vi "AlliGator with Tabs Register Control Events.vi"(8 "Error In":errorcluster) -> (0 "Error Out":errorcluster, 3 "AlliGator Events Registration":T1)   [LabVIEW 2021, in "AlliGator GUI.lvlib"]
doc: "Registers user events for controls on the main AlliGator window."
uses:
  AlliGator GUI.lvlib
  Settings/AlliGator Settings+.lvlib
  Phasor Plot Color Map/AlliGator Phasor Plot Color Map.lvlib
  Graphs/XY Graph/XY Graph Add-Ons.lvlib
  Decay Graph/AlliGator Decay Graph.lvlib
  Intensity Time Trace/AlliGator Intensity Time Trace.lvlib
  Decay Statistics/AlliGator Decay Statistics.lvlib
  Phasor Graph/AlliGator Phasor Graph.lvlib
  Phasor Ratio/AlliGator Phasor Ratio.lvlib
  Lifetime & Other Parameters/AlliGator Lifetime & Other Parameters.lvlib
  Settings/AlliGator Settings Window Messages.ctl
  Settings/AlliGator Settings Event.ctl
  Phasor Plot Color Map/AlliGator Phasor Color Map User Event List.ctl
  AlliGator Subpanel Event Data.ctl
  Graphs/XY Graph/XY Graph Refnum.ctl
  AlliGator with Tabs Events Registration.ctl
  Phasor Plot/AlliGator Phasor Plot.lvlib
  Decay Fit Parameter Map/AlliGator Decay Fit Parameter Map.lvlib
  Parameter Map/AlliGator Parameter Map.lvlib
panel:
  # "see the AlliGator License on the block diagram (Ctrl+E or Window:Show Block Diagram)"
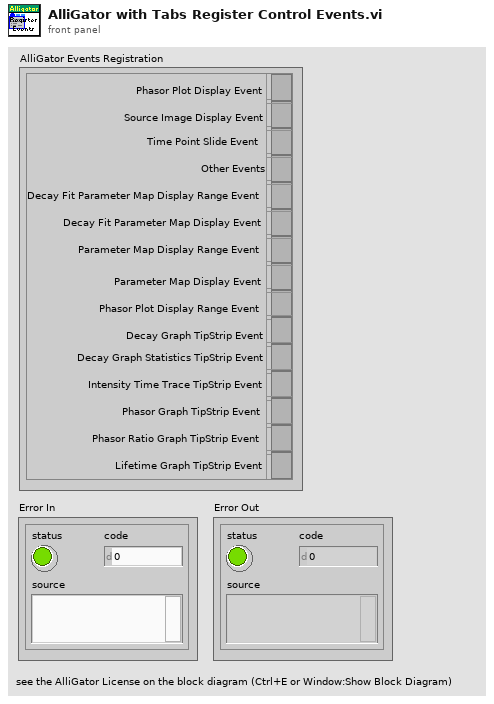
[diagram p1: front panel]
types:
  T1 = typedef "AlliGator GUI.lvlib/AlliGator with Tabs Events Registration.ctl" = cluster{"Phasor Plot Display Event":refnum<event-registration>, "Source Image Display Event":refnum<event-registration>, "Time Point Slide Event":refnum<event-registration>, "Other Events":refnum<event-registration>, "Decay Fit Parameter Map Display Range Event":refnum<event-registration>, "Decay Fit Parameter Map Display Event":refnum<event-registration>, "Parameter Map Display Range Event":refnum<event-registration>, "Parameter Map Display Event":refnum<event-registration>, "Phasor Plot Display Range Event":refnum<event-registration>, "Decay Graph TipStrip Event":refnum<event-registration>, "Decay Graph Statistics TipStrip Event":refnum<event-registration>, "Intensity Time Trace TipStrip Event":refnum<event-registration>, "Phasor Graph TipStrip Event":refnum<event-registration>, "Phasor Ratio Graph TipStrip Event":refnum<event-registration>, "Lifetime Graph TipStrip Event":refnum<event-registration>}
  T2 = typedef "AlliGator Decay Graph.lvlib/AlliGator Decay Graph Ctrl Refnums.ctl" = cluster{"Decay Graph":refnum<vi>, "Decay Graph Active":refnum<vi>, "Decay Background":refnum<vi>, "Decay Integrated Intensity":refnum<vi>, "Decay Lifetime":refnum<vi>}
  T3 = typedef "AlliGator Decay Statistics.lvlib/AlliGator Decay Statistics Graph Ctrl Refnums.ctl" = cluster{"Decay Statistics Graph":refnum<vi>, "Decay Statistics Bin":refnum<vi>}
  T4 = typedef "AlliGator Intensity Time Trace.lvlib/AlliGator Intensity Time Trace Ctrl Refnums.ctl" = cluster{"Intensity Time Trace":refnum<vi>, "Time Step":refnum<vi>, "Use File Timestamp":refnum<vi>}
  T5 = typedef "AlliGator Phasor Graph.lvlib/AlliGator Phasor Graph Ctrl Refnums.ctl" = cluster{"Phasor Ratio":refnum<vi>, "Modulus Lifetime":refnum<vi>, "Phasor at cursor (m, phi)":refnum<vi>, "Phase Lifetime":refnum<vi>, "Phasor at cursor (g, s)":refnum<vi>, "Phasor Graph Average Lifetime":refnum<vi>, "Phasor Graph Active":refnum<vi>, "Save Phasor Graph":refnum<vi>, "Phasor Frame Slide":refnum<vi>, "Single Step Phasor":refnum<vi>, "Calibration Type":refnum<vi>, "Show Line":refnum<vi>, "Phase Lifetime 1":refnum<vi>, "Phase Lifetime 2":refnum<vi>, "Phasor Graph Frequency":refnum<vi>, "Phasor Reference 1 Control":refnum<vi>, "Phasor Reference 2 Control":refnum<vi>, "Calibration Lifetime":refnum<vi>, "Phase Lifetime SDV":refnum<vi>, "Average Lifetime SDV":refnum<vi>, "Phasor Ratio SDV":refnum<vi>, "Modulus Lifetime SDV":refnum<vi>, "Phasor Graph":refnum<vi>}
  T6 = typedef "AlliGator Phasor Ratio.lvlib/AlliGator Phasor Ratio Graph Ctrl Refnums.ctl" = cluster{"Phasor Ratio Graph":refnum<vi>}
  T7 = typedef "AlliGator Lifetime & Other Parameters.lvlib/AlliGator Lifetime & Other Parameters Ctrl Refnums.ctl" = cluster{"Lifetime Graph":refnum<vi>}
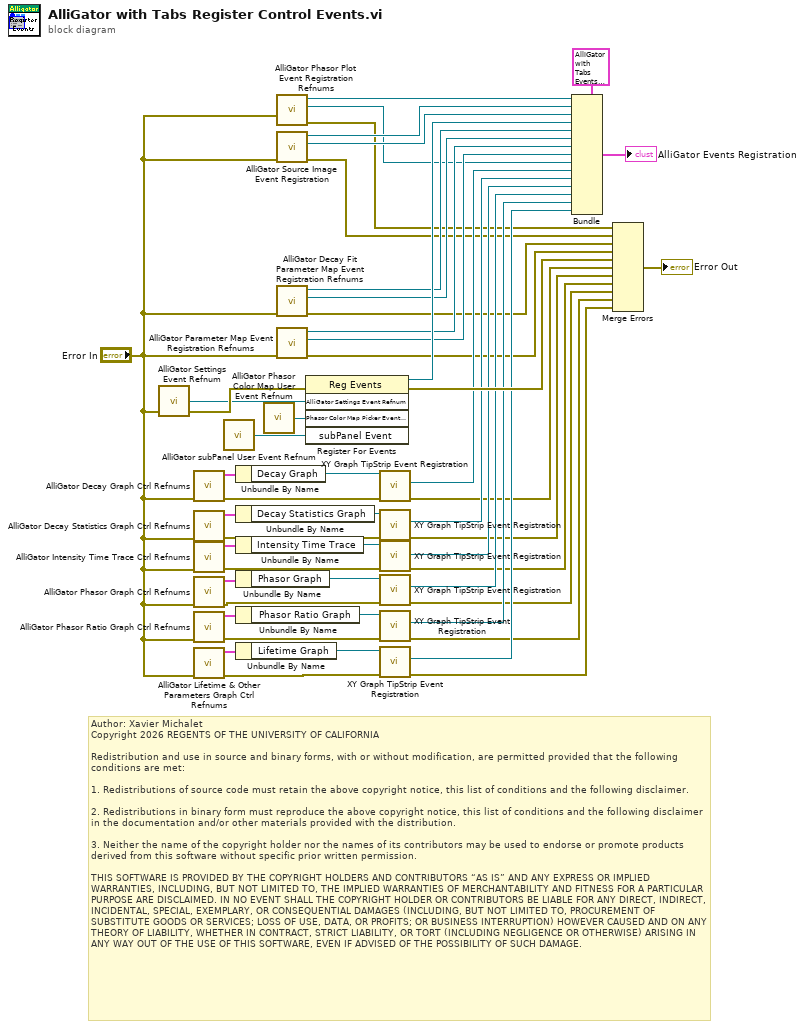
[diagram p0: block diagram]
diagram:
  # "Author: Xavier Michalet\nCopyright 2026 REGENTS OF THE UNIVERSITY OF CALIFORNIA\n\nRedistribution and use in source and binary forms, with or without modification, are permitted provided that the following conditions are met:\n\n1. Redistributions of source code must retain the above copyright notice, this list of conditions and the following disclaimer.\n\n2. Redistributions in binary form must reproduce the above copyright notice, this list of conditions and the following disclaimer in the documentation and/or other materials provided with the distribution.\n\n3. Neither the name of the copyright holder nor the names of its contributors may be used to endorse or promote products derived from this software without specific prior written permission.\n\nTHIS SOFTWARE IS PROVIDED BY THE COPYRIGHT HOLDERS AND CONTRIBUTORS “AS IS” AND ANY EXPRESS OR IMPLIED WARRANTIES, INCLUDING, BUT NOT LIMITED TO, THE IMPLIED WARRANTIES OF MERCHANTABILITY AND FITNESS FOR A PARTICULAR PURPOSE ARE DISCLAIMED. IN NO EVENT SHALL THE COPYRIGHT HOLDER OR CONTRIBUTORS BE LIABLE FOR ANY DIRECT, INDIRECT, INCIDENTAL, SPECIAL, EXEMPLARY, OR CONSEQUENTIAL DAMAGES (INCLUDING, BUT NOT LIMITED TO, PROCUREMENT OF SUBSTITUTE GOODS OR SERVICES; LOSS OF USE, DATA, OR PROFITS; OR BUSINESS INTERRUPTION) HOWEVER CAUSED AND ON ANY THEORY OF LIABILITY, WHETHER IN CONTRACT, STRICT LIABILITY, OR TORT (INCLUDING NEGLIGENCE OR OTHERWISE) ARISING IN ANY WAY OUT OF THE USE OF THIS SOFTWARE, EVEN IF ADVISED OF THE POSSIBILITY OF SUCH DAMAGE."
  n1 = call "AlliGator Settings Event Refnum.vi"("Error In"="Error In") -> ("AlliGator Settings Event Refnum"=w11:refnum<user-event>, "Error Out"=w45:errorcluster)  [unwired: 7 in]
  n2 = call "AlliGator Decay Graph Ctrl Refnums.vi"("error in (no error)"="Error In") -> ("error out"=w23:errorcluster, "Decay Graph Ctrl Refnums"=w35:T2)  [unwired: 9 in]
  n3 = call "AlliGator Decay Statistics Graph Ctrl Refnums.vi"("error in (no error)"="Error In") -> ("error out"=w22:errorcluster, "Decay Statistics Graph Ctrl Refnums"=w31:T3)  [unwired: 9 in]
  n4 = call "AlliGator Intensity Time Trace Ctrl Refnums.vi"("error in (no error)"="Error In") -> ("error out"=w21:errorcluster, "Intensity Time Trace Ctrl Refnums"=w33:T4)  [unwired: 9 in]
  n5 = call "AlliGator Phasor Graph Ctrl Refnums.vi"("error in (no error)"="Error In") -> ("error out"=w20:errorcluster, "Phasor Graph Ctrl Refnums"=w29:T5)  [unwired: 9 in]
  n6 = call "AlliGator Phasor Ratio Graph Ctrl Refnums.vi"("error in (no error)"="Error In") -> ("error out"=w19:errorcluster, "Phasor Ratio Graph Ctrl Refnums"=w27:T6)  [unwired: 9 in]
  n7 = call "AlliGator Lifetime & Other Parameters Graph Ctrl Refnums.vi"("error in (no error)"="Error In") -> ("error out"=w18:errorcluster, "Lifetime & Other Parameters Graph Ctrl Refnums"=w25:T7)  [unwired: 9 in]
  n8 = call "AlliGator subPanel User Event Refnum.vi"() -> ("subPanel Event"=w49:refnum<user-event>)  [unwired: 9 in]
  n9 = Unbundle By Name(w35) -> ("Decay Graph"=w34:refnum<vi>)
  n10 = Unbundle By Name(w31) -> ("Decay Statistics Graph"=w30:refnum<vi>)
  n11 = Unbundle By Name(w33) -> ("Intensity Time Trace"=w32:refnum<vi>)
  n12 = Unbundle By Name(w29) -> ("Phasor Graph"=w28:refnum<vi>)
  n13 = Unbundle By Name(w27) -> ("Phasor Ratio Graph"=w26:refnum<vi>)
  n14 = Unbundle By Name(w25) -> ("Lifetime Graph"=w24:refnum<vi>)
  n15 = call "AlliGator Phasor Color Map User Event Refnum.vi"() -> ("Phasor Color Map Picker Event Refnum"=w50:refnum<user-event>)  [unwired: 9 in]
  n16 = call "AlliGator Phasor Plot Event Registration Refnums.vi"("error in (no error)"="Error In") -> ("error out"=w1:errorcluster, "Phasor Plote Display Range Event"=w6:refnum<event-registration>, "Phasor Plot Display Event"=w9:refnum<event-registration>)  [unwired: 8 in]
  n17 = call "AlliGator Source Image Event Registration.vi"("error in (no error)"="Error In") -> ("error out"=w3:errorcluster, "Time Point Slide Event Registration"=w46:refnum<event-registration>, "Source Image Display Event Registration"=w51:refnum<event-registration>)  [unwired: 8 in]
  n18 = call "AlliGator Decay Fit Parameter Map Event Registration Refnums.vi"("error in (no error)"="Error In") -> ("error out"=w4:errorcluster, "Decay Fit Parameter Map Display Event"=w43:refnum<event-registration>, "Decay Fit Parameter Map Display Range Event"=w44:refnum<event-registration>)  [unwired: 8 in]
  n19 = call "AlliGator Parameter Map Event Registration Refnums.vi"("error in (no error)"="Error In") -> ("error out"=w5:errorcluster, "Parameter Map Display Event"=w7:refnum<event-registration>, "Parameter Map Display Range Event"=w8:refnum<event-registration>)  [unwired: 8 in]
  n20 = register-events(error in=w45, w11, w50, w49) -> (reference out=w48:refnum<event-registration>, error out=w47:errorcluster)  [unwired: 1 in]
  n21 = call "XY Graph TipStrip Event Registration.vi"("error in (no error)"=w23, "XY Graph Refnum"=w34) -> ("error out"=w17:errorcluster, "Event Registration Refnum"=w42:refnum<event-registration>)  [unwired: 7 in, 1 out]
  n22 = call "XY Graph TipStrip Event Registration.vi"("error in (no error)"=w22, "XY Graph Refnum"=w30) -> ("error out"=w16:errorcluster, "Event Registration Refnum"=w40:refnum<event-registration>)  [unwired: 7 in, 1 out]
  n23 = call "XY Graph TipStrip Event Registration.vi"("error in (no error)"=w21, "XY Graph Refnum"=w32) -> ("error out"=w15:errorcluster, "Event Registration Refnum"=w39:refnum<event-registration>)  [unwired: 7 in, 1 out]
  n24 = call "XY Graph TipStrip Event Registration.vi"("error in (no error)"=w20, "XY Graph Refnum"=w28) -> ("error out"=w14:errorcluster, "Event Registration Refnum"=w38:refnum<event-registration>)  [unwired: 7 in, 1 out]
  n25 = call "XY Graph TipStrip Event Registration.vi"("error in (no error)"=w19, "XY Graph Refnum"=w26) -> ("error out"=w13:errorcluster, "Event Registration Refnum"=w37:refnum<event-registration>)  [unwired: 7 in, 1 out]
  n26 = call "XY Graph TipStrip Event Registration.vi"("error in (no error)"=w18, "XY Graph Refnum"=w24) -> ("error out"=w12:errorcluster, "Event Registration Refnum"=w36:refnum<event-registration>)  [unwired: 7 in, 1 out]
  n27 = Bundle(cluster=T1 {"Phasor Plot Display Event"=refnum, "Source Image Display Event"=refnum, "Time Point Slide Event"=refnum, "Other Events"=refnum, "Decay Fit Parameter Map Display Range Event"=refnum, "Decay Fit Parameter Map Display Event"=refnum, "Parameter Map Display Range Event"=refnum, "Parameter Map Display Event"=refnum, "Phasor Plot Display Range Event"=refnum, "Decay Graph TipStrip Event"=refnum, "Decay Graph Statistics TipStrip Event"=refnum, "Intensity Time Trace TipStrip Event"=refnum, "Phasor Graph TipStrip Event"=refnum, "Phasor Ratio Graph TipStrip Event"=refnum, "Lifetime Graph TipStrip Event"=refnum} ("AlliGator Events Registration"), "Phasor Plot Display Event"=w9, "Source Image Display Event"=w51, "Time Point Slide Event"=w46, "Other Events"=w48, "Decay Fit Parameter Map Display Range Event"=w44, "Decay Fit Parameter Map Display Event"=w43, "Parameter Map Display Range Event"=w8, "Parameter Map Display Event"=w7, "Phasor Plot Display Range Event"=w6, "Decay Graph TipStrip Event"=w42, "Decay Graph Statistics TipStrip Event"=w40, "Intensity Time Trace TipStrip Event"=w39, "Phasor Graph TipStrip Event"=w38, "Phasor Ratio Graph TipStrip Event"=w37, "Lifetime Graph TipStrip Event"=w36) -> (→"AlliGator Events Registration":T1)
  n28 = Merge Errors(w1, w3, w4, w5, w47, w17, w16, w15, w14, w13, w12) -> (→"Error Out":errorcluster)
